vi "When Delete.vi"(0 "error out":errorcluster, 11 "IFile Manager in":refnum<class "Mock IFile Manager.lvclass">) -> (3 "IFile Manager out":refnum<class "Mock IFile Manager.lvclass">)   [LabVIEW 2026, in "Mock IFile Manager.lvclass"]
doc: "Delete a file or folder without prompts."
uses:
  Mock IFile Manager.lvclass
  Mock IFile Manager.lvclass/Mock IFile Manager.ctl
  C:/Program Files/National Instruments/LabVIEW 2026/vi.lib/Astemes/LMock/Mock.lvclass
  C:/Users/juanj/Documents/hasbun_wood_engineering/github/py2vi/labview/Mocks/Mock IFile Manager/Mock IFile Manager.lvclass
  C:/Users/juanj/Documents/hasbun_wood_engineering/github/py2vi/labview/Interfaces/IFile Manager/IFile Manager.lvclass
  <vilib>/Astemes/LMock/Mock.lvclass
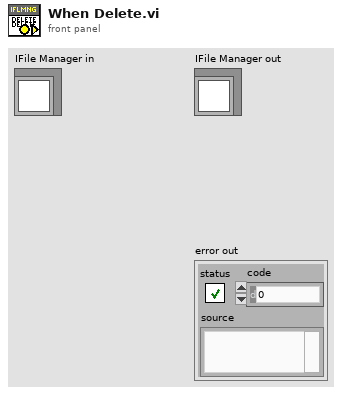
[diagram p1: front panel]
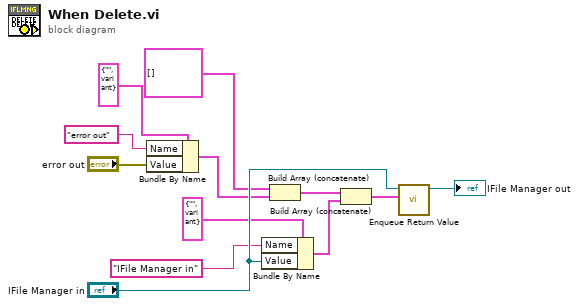
[diagram p0: block diagram]
diagram:
  n1 = Bundle By Name(cluster=cluster{"Name":string, "Value":variant} {"Name"="", "Value"=variant} ("element"), "Name"="error out", "Value"="error out") -> (w3:cluster{"Name":string, "Value":variant})
  n2 = Bundle By Name(cluster=cluster{"Name":string, "Value":variant} {"Name"="", "Value"=variant} ("element"), "Name"="IFile Manager in", "Value"="IFile Manager in") -> (w1:cluster{"Name":string, "Value":variant})
  n3 = Build Array (concatenate)(cluster{"Name":string, "Value":variant}[] [] ("Control Values"), w3) -> (w8:cluster{"Name":string, "Value":variant}[])
  n4 = Build Array (concatenate)(w8, w1) -> (w10:cluster{"Name":string, "Value":variant}[])
  n5 = call <vilib>:"Enqueue Return Value.vi"("Indicator Values"=w10, "Mock In"="IFile Manager in") -> ("Mock Out"=→"IFile Manager out":refnum<class "Mock IFile Manager.lvclass">)  [unwired: 8 in, 1 out]
